vi "Create.vi"(5 "Class in":refnum<class "Class.lvclass">, 8 "error in (no error)":errorcluster, 10 "Filename":path, 11 "Name":string) -> (0 "error out":errorcluster, 3 "Class":refnum<class "Class.lvclass">)   [LabVIEW 2017, in "Cobertura.lvlib" / "Class.lvclass"]
uses:
  Class.lvclass
  Class.lvclass/Class.ctl
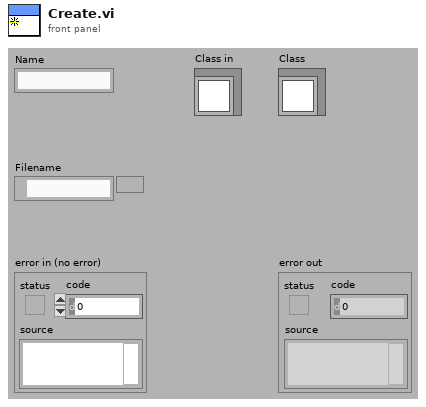
[diagram p1: front panel]
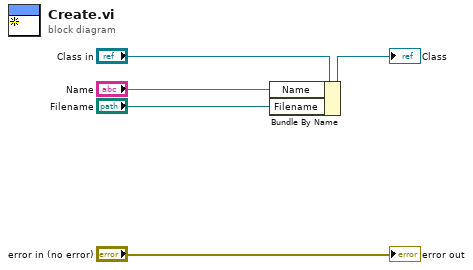
[diagram p0: block diagram]
diagram:
  n1 = Bundle By Name(cluster="Class in", "Name"="Name", "Filename"="Filename") -> (→"Class":refnum<class "Class.lvclass">)
  "error out" <- "error in (no error)"
